vi "VIH Utility - FILE - List Directory.vi"(8 "error in":errorcluster, 10 "patterns":string[](array[string]), 11 "directory path":path) -> (0 "error out":errorcluster, 1 "directory paths":path[](array[path]), 2 "file paths":path[](array[path]), 3 "dup directory path":path)   [LabVIEW 2014]
doc: "::: VI Helpeks :::\nCopyright (c) 2000-2026 Konstantin Shifershteyn. All rights reserved."
panel:
  # "VI Helpeks\nCopyright (c) 2012-2026 Konstantin Shifershteyn"
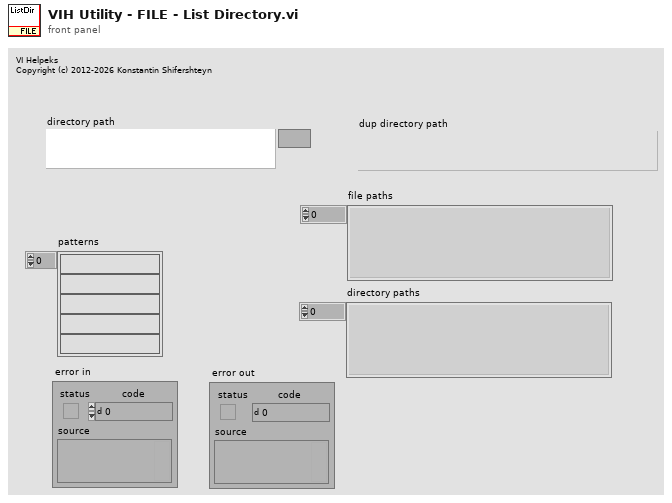
[diagram p1: front panel]
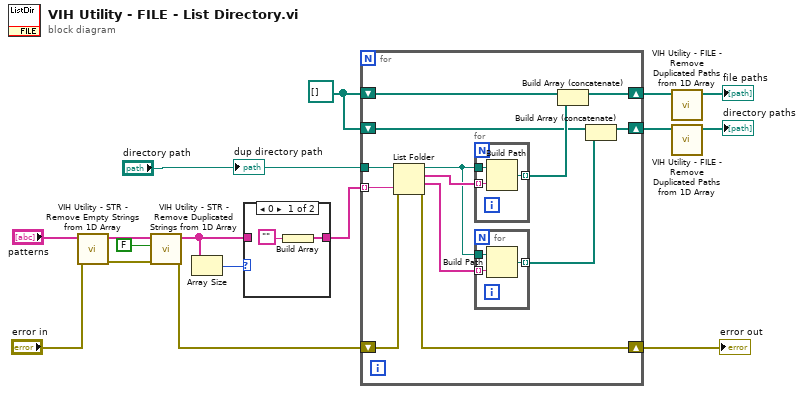
[diagram p0: block diagram]
diagram:
  w14 = path[] []
  n1 = call "VIH Utility - STR - Remove Empty Strings from 1D Array.vi"("error in"="error in", "String array in"="patterns") -> ("error out"=w3:errorcluster, "String array out"=w7:string[])  [unwired: 8 in]
  n2 = call "VIH Utility - STR - Remove Duplicated Strings from 1D Array.vi"("error in (no error)"=w3, "case sensitive comparison (T)"=FALSE, "Array in"=w7) -> ("error out"=w2:errorcluster, "Array out"=w6:string[])  [unwired: 7 in]
  n3 = Array Size(array=w6) -> (size(s)=w16:i32)
  n4 = case shown="0" w16 {
    tunnel: w6 -> [_ w19]
    tunnel: [w18 w19] -> w15
    frame 0 {
      n5 = Build Array("") -> (w18:string[])
    }
    frame 1, Default {
    }
  }
  n6 = for {
    tunnel: "directory path" -> [w32]
    shift-right: [w30] -> w13
    shift-left: w2 -> [w31]
    shift-right: [w28] -> w11
    shift-left: w14 -> [w29]
    tunnel: w15 -> [w26] mode=indexing
    shift-right: [w25] -> w9
    shift-left: w14 -> [w24]
    n7 = List Folder(path=w32, pattern=w26, error in=w31) -> (path out=w22:path, filenames=w23:string[], folder names=w21:string[], error out=w30:errorcluster)  [unwired: 1 out]
    n8 = for {
      tunnel: w22 -> [w38]
      tunnel: w23 -> [w37] mode=indexing
      tunnel: [w36] -> w27 mode=indexing
      n9 = Build Path(base path=w38, name or relative path=w37) -> (appended path=w36:path)
    }
    n10 = for {
      tunnel: w22 -> [w35]
      tunnel: w21 -> [w34] mode=indexing
      tunnel: [w33] -> w20 mode=indexing
      n11 = Build Path(base path=w35, name or relative path=w34) -> (appended path=w33:path)
    }
    n12 = Build Array (concatenate)(w29, w27) -> (w28:path[])
    n13 = Build Array (concatenate)(w24, w20) -> (w25:path[])
  }
  "error out" <- w13
  n14 = call "VIH Utility - FILE - Remove Duplicated Paths from 1D Array.vi"("Array in"=w11) -> ("Array out"=→"file paths":path[])  [unwired: 9 in, 1 out]
  n15 = call "VIH Utility - FILE - Remove Duplicated Paths from 1D Array.vi"("Array in"=w9) -> ("Array out"=→"directory paths":path[])  [unwired: 9 in, 1 out]
  "dup directory path" <- "directory path"
